vi "Convert CAN frames to Trace log.vi"(11 "can frames in":T1[](array[typedef]) {"payload" format="%x"; "timestamp" format="%<%.7X\n%x>T"; "type" items=["CAN Data"=0, "CAN Remote"=1, "CAN Bus Error"=2, "CAN 2.0 Data"=8, "CAN FD Data"=16, "CAN FD+BRS Data"=24, "J1939 Data"=192, "Delay"=224, "Log Trigger"=225, "Start Trigger"=226]; "identifier" format="%x"}) -> (3 "trace out":string[][](array[string]))   [LabVIEW 2025, in "CAN-LIN Raw Bus Capture.lvclass"]
uses:
  CAN-LIN Raw Bus Capture.lvclass
  <vilib>/xnet/xnet.llb/XNET Frame CAN.ctl
  <vilib>/xnet/xnet.llb/XNET Frame Type CAN.ctl
  <vilib>/Utility/error.llb/Trim Whitespace One-Sided.vi
  CAN-LIN Raw Bus Capture.lvclass/CAN-LIN Raw Bus Capture.ctl
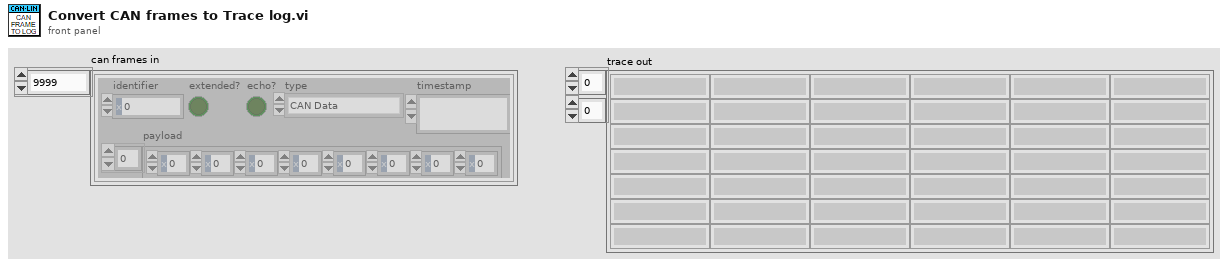
[diagram p1: front panel]
types:
  T1 = typedef "XNET Frame CAN.ctl" = cluster{"timestamp":timestamp, "payload":u8[], "identifier":u32, "type":T2, "extended?":bool, "echo?":bool}
  T2 = typedef "XNET Frame Type CAN.ctl" = u8
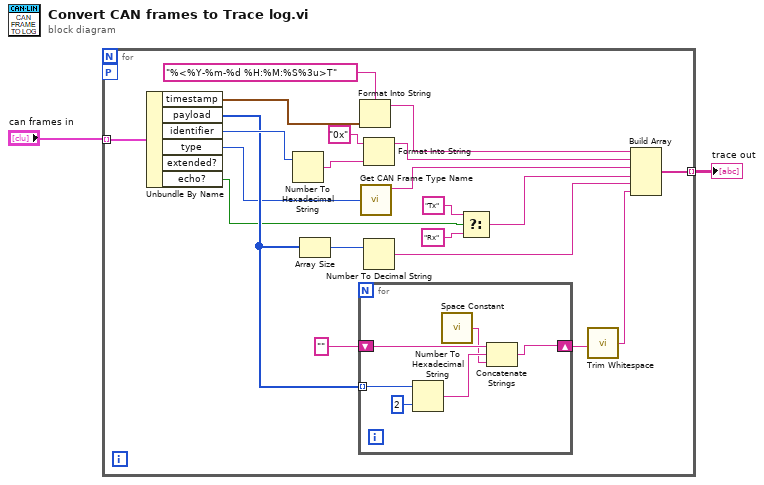
[diagram p0: block diagram]
diagram:
  n1 = for {
    tunnel: "can frames in" -> [w23] mode=indexing
    tunnel: [w21] -> w1 mode=indexing
    workers-P: _ -> [_]
    n2 = Unbundle By Name(w23) -> ("timestamp"=w20:timestamp, "payload"=w16:u8[], "identifier"=w22:u32, "type"=w14:T2, "echo?"=w8:bool)  [unwired: 1 out]
    n3 = Number To Hexadecimal String(2:w22) -> (0:w4:string)  [unwired: 1 in]
    n4 = Array Size(array=w16) -> (size(s)=w17:i32)
    n5 = for {
      tunnel: w16 -> [w29] mode=indexing
      shift-right: [w26] -> w12
      shift-left: "" ("format string") -> [w28]
      n6 = Number To Hexadecimal String(1:i16 2 ("width (-)"), 2:w29) -> (0:w27:string)
      n7 = call <vilib>:"Space Constant.vi"() -> ("String"=w24:string)
      n8 = Concatenate Strings(w28, w27, w24) -> (w26:string)
    }
    n9 = Format Into String(format string="%<%Y-%m-%d %H:%M:%S%3u>T", w20) -> (resulting string=w19:string)  [unwired: 2 in, 1 out]
    n10 = call "Get CAN Frame Type Name.vi"("can frame type id"=w14) -> ("can frame type name"=w13:string)  [unwired: 10 in]
    n11 = Format Into String(initial string="0x", w4) -> (resulting string=w3:string)  [unwired: 2 in, 1 out]
    n12 = Number To Decimal String(number=w17) -> (decimal integer string=w11:string)  [unwired: 1 in]
    n13 = Select(t="Tx" ("format string"), s=w8, f="Rx" ("format string")) -> (s? t:f=w7:string)
    n14 = call <vilib>:"Trim Whitespace.vi"("string"=w12) -> ("trimmed string"=w6:string)  [unwired: 1 in]
    n15 = Build Array(w19, w3, w13, w7, w11, w6) -> (w21:string[])
  }
  "trace out" <- w1
